vi "Reset Hardware List and Run Button.vi"(8 "error in (no error)":errorcluster, 11 "Measurement UI in":refnum<class "Measurement UI.lvclass">) -> (0 "error out":errorcluster, 3 "Measurement UI out":refnum<class "Measurement UI.lvclass">)   [LabVIEW 2017, in "Measurement UI.lvlib" / "Measurement UI.lvclass"]
uses:
  Measurement UI.lvclass
  Measurement UI.lvclass/Measurement UI.ctl
  Accessors/Read Show FP_.vi
  Accessors/Read Run.vi
  Accessors/Read Digitizer.vi
  Read Multimeter.vi
  Accessors/Read Function Generator.vi
  Accessors/Read Power Supply.vi
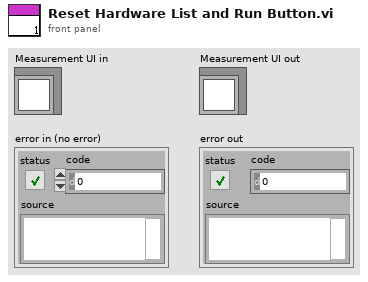
[diagram p1: front panel]
types:
  T1 = enum8{"Enabled", "Disabled", "Disabled and Grayed Out"}
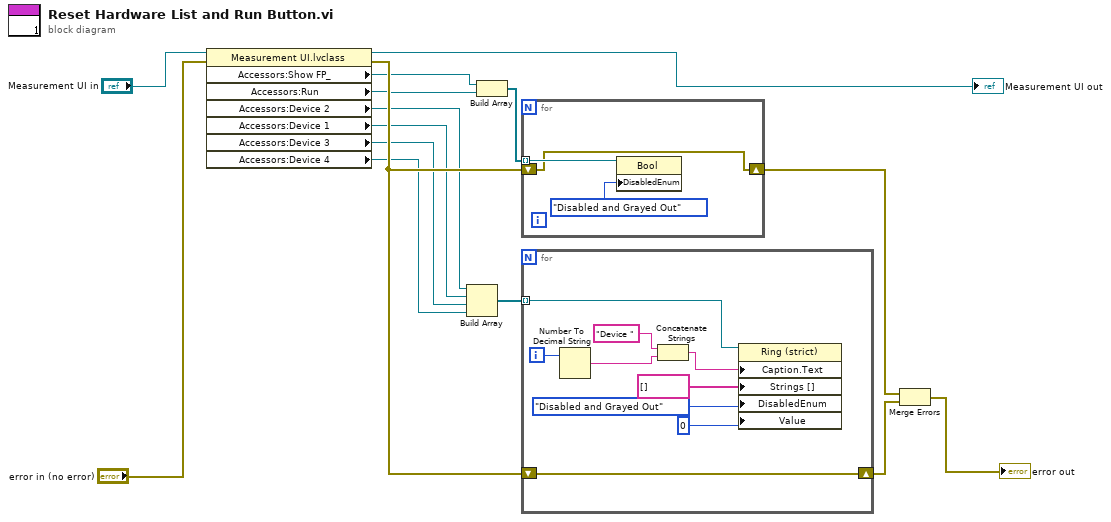
[diagram p0: block diagram]
diagram:
  n1 = property class="Measurement UI.lvclass"(reference="Measurement UI in", error in="error in (no error)") -> (reference out=→"Measurement UI out":refnum<class "Measurement UI.lvclass">, error out=w12:errorcluster, "Accessors:Show FP_"=w1:refnum<vi>, "Accessors:Run"=w3:refnum<vi>, "Accessors:Device 2"=w6:refnum<vi>, "Accessors:Device 1"=w7:refnum<vi>, "Accessors:Device 3"=w8:refnum<vi>, "Accessors:Device 4"=w9:refnum<vi>)
  n2 = Build Array(w6, w7, w8, w9) -> (w4:refnum<vi>[])
  n3 = Build Array(w1, w3) -> (w2:refnum<vi>[])
  n4 = for {
    tunnel: w2 -> [w18] mode=indexing
    shift-right: [w16] -> w14
    shift-left: w12 -> [w16]
    n5 = property class="Bool"(reference=w18, "DisabledEnum"=T1."Disabled and Grayed Out" ("Disabled")) -> ()  [unwired: 1 in, 2 out]
  }
  n6 = for {
    tunnel: w4 -> [w24] mode=indexing
    shift-right: [w19] -> w13
    shift-left: w12 -> [w19]
    i -> [w23]
    n7 = Number To Decimal String(number=w23) -> (decimal integer string=w21:string)  [unwired: 1 in]
    n8 = Concatenate Strings("Device ", w21) -> (w20:string)
    n9 = property class="Ring (strict)"(reference=w24, "Caption.Text"=w20, "Strings []"=string[] [], "DisabledEnum"=T1."Disabled and Grayed Out" ("Disabled"), "Value"=u16 0) -> ()  [unwired: 1 in, 2 out]
  }
  n10 = Merge Errors(w14, w13) -> (→"error out":errorcluster)
